vi "Write Signals.vi"(8 "error in (no error)":errorcluster, 9 "DO Finite Pulse Config":T1={"Port Number"=0, "Number of Pulses"=20, "High Time (ms)"=20, "Low Time (ms)"=20}, 10 "Command DO Pulse":bool, 11 "session in":refnum<k21>) -> (0 "error out":errorcluster, 3 "session out":refnum<k21>)   [LabVIEW 2023]
uses:
  <vilib>/xnet/xnet.llb/XNET Write (Signal Single-point).vi
  DUT Sample/typedefs/DO Finite Pulse Config.ctl
  DUT Sample/DUT Sample.lvclass
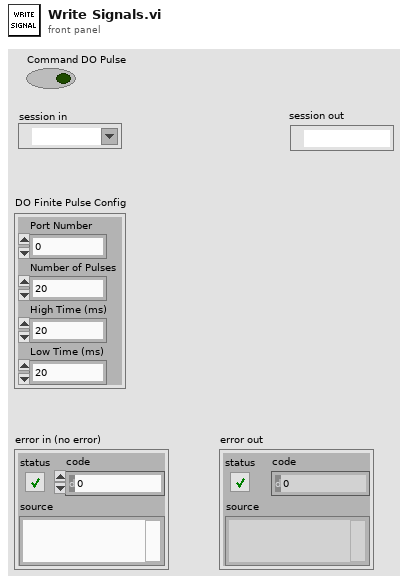
[diagram p1: front panel]
types:
  T1 = typedef "DUT Sample.lvclass/DO Finite Pulse Config.ctl" = cluster{"Port Number":u8, "Number of Pulses":u8, "High Time (ms)":u16, "Low Time (ms)":u16}
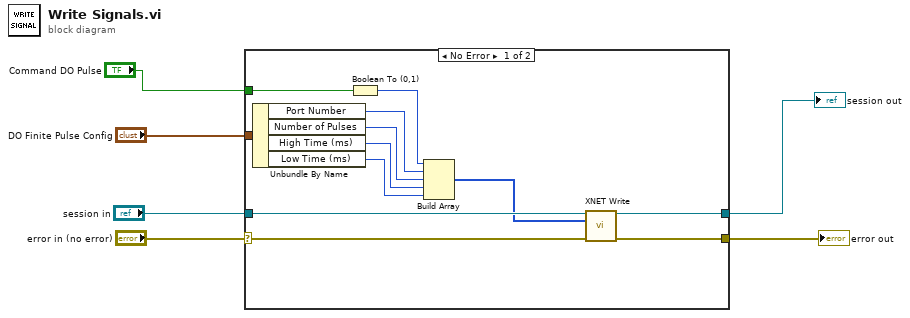
[diagram p0: block diagram]
diagram:
  n1 = case shown="No Error" "error in (no error)" {
    selector: "error in (no error)" -> [w11 w19]
    tunnel: "session in" -> [w18 _]
    tunnel: "DO Finite Pulse Config" -> [w17 _]
    tunnel: [w10 w19] -> w3
    tunnel: [w9 _] -> w2
    tunnel: "Command DO Pulse" -> [w8 _]
    frame No Error {
      n2 = Unbundle By Name(w17) -> ("Port Number"=w16:u8, "Number of Pulses"=w15:u8, "High Time (ms)"=w14:u16, "Low Time (ms)"=w13:u16)
      n3 = Boolean To (0,1)(Boolean=w8) -> (0, 1=w7:i16)
      n4 = Build Array(w7, w16, w15, w14, w13) -> (w12:u16[])
      n5 = call-poly <vilib>:"XNET Write.vi"("session in"=w18, "data"=w12, "error in (no error)"=w11) -> ("session out"=w9:refnum<k21>, "error out"=w10:errorcluster)  [unwired: 11 in]
    }
    frame Error {
    }
  }
  "error out" <- w3
  "session out" <- w2
